vi "Create Signal Properties - Sine.vi"(8 "error in (no error)":errorcluster, 10 "sine wave properties":T1, 11 "AudioGeneration in":refnum<class "AudioGeneration.lvclass">) -> (0 "error out":errorcluster, 2 "signal settings":T2, 3 "AudioGeneration out":refnum<class "AudioGeneration.lvclass">)   [LabVIEW 2021, in "AudioGeneration.lvclass"]
uses:
  AudioGeneration.lvclass
  AudioGeneration.lvclass/AudioGeneration.ctl
  controls/signal type.ctl
  controls/AudioGenTypeDefs.lvlib
  controls/signal settings.ctl
  controls/sine wave properties.ctl
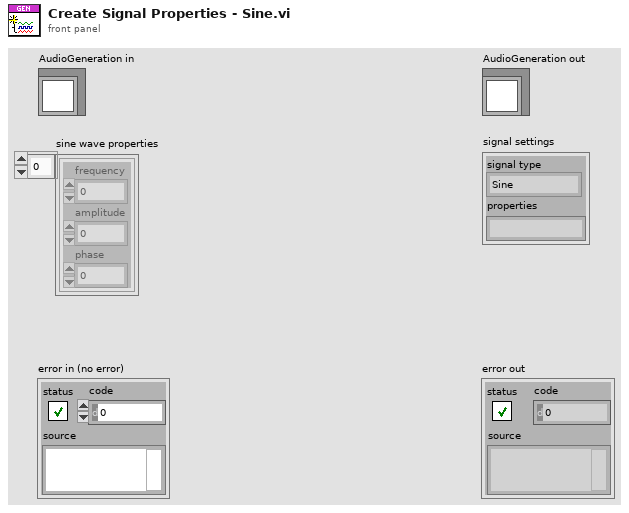
[diagram p1: front panel]
types:
  T1 = typedef "AudioGenTypeDefs.lvlib/sine wave properties.ctl" = cluster{"frequency":dbl, "amplitude":dbl, "phase":dbl}[]
  T2 = typedef "AudioGenTypeDefs.lvlib/signal settings.ctl" = cluster{"signal type":T3, "properties":string}
  T3 = typedef "AudioGenTypeDefs.lvlib/signal type.ctl" = enum16{"Sine", "Square", "Triangle", "White Noise", "Pink Noise", "Periodic Random Noise"}
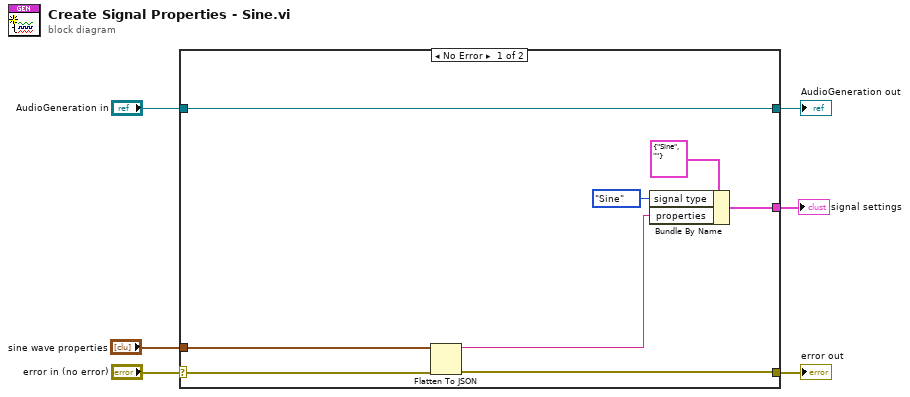
[diagram p0: block diagram]
diagram:
  n1 = case shown="No Error" "error in (no error)" {
    selector: "error in (no error)" -> [w10 w16]
    tunnel: [w8 w16] -> w5
    tunnel: [w14 w15] -> w3
    tunnel: "AudioGeneration in" -> [w14 w15]
    tunnel: [w12 _] -> w2
    tunnel: "sine wave properties" -> [w7 _]
    frame No Error {
      n2 = Flatten To JSON(anything=w7, error in (no error)=w10) -> (JSON string=w9:string, 11:w8:errorcluster)  [unwired: 1 in]
      n3 = Bundle By Name(cluster=T2 {"signal type"=enum."Sine", "properties"=""} ("signal settings"), "signal type"=signal_type."Sine", "properties"=w9) -> (w12:T2)
    }
    frame Error {
    }
  }
  "error out" <- w5
  "AudioGeneration out" <- w3
  "signal settings" <- w2
